vi "VIH ProjFile - XML - Text Node - Create.vi"(8 "error in":errorcluster, 10 "Data":string, 11 "XML Parent Item":refnum<k20>) -> (0 "error out":errorcluster, 3 "dup XML Parent Item":refnum<k20>)   [LabVIEW 2014]
doc: "::: VI Helpeks :::\nCopyright (c) 2000-2026 Konstantin Shifershteyn. All rights reserved."
uses:
  <vilib>/xml/Close Reference(Node).vi
  <resource>/objmgr/DOMUserDefRef.rc
  <vilib>/xml/NI_XML.lvlib
panel:
  # "VI Helpeks\nCopyright (c) 2012-2026 Konstantin Shifershteyn"
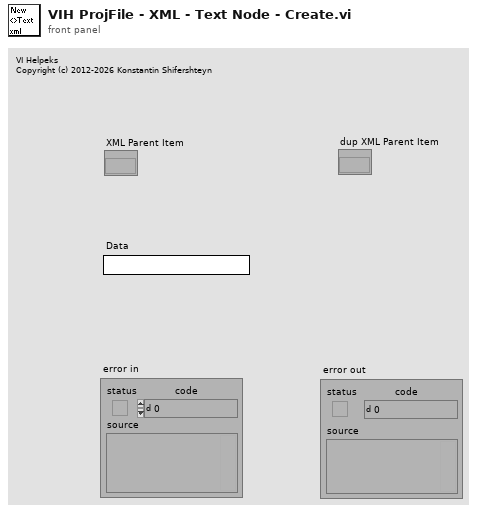
[diagram p1: front panel]
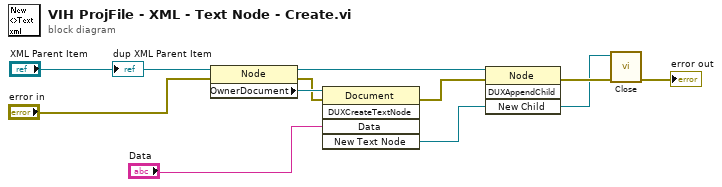
[diagram p0: block diagram]
diagram:
  n1 = property class="Node"(reference="XML Parent Item", error in="error in") -> (reference out=w8:refnum<k20>, error out=w7:errorcluster, "OwnerDocument"=w9:refnum<k20>)
  n2 = invoke class="Document" method="DUXCreateTextNode"(reference=w9, error in=w7, "Data"="Data") -> (error out=w5:errorcluster, "New Text Node"=w2:refnum<k20>)  [unwired: 2 in, 3 out]
  n3 = invoke class="Node" method="DUXAppendChild"(reference=w8, error in=w5, "New Child"=w2) -> (error out=w4:errorcluster)  [unwired: 1 in, 3 out]
  n4 = call-poly <vilib>:"Close.vi"("error in (no error)"=w4, "node"=w2) -> ("error out"=→"error out":errorcluster)  [unwired: 7 in]
  "dup XML Parent Item" <- "XML Parent Item"
